vi "PicoScope3000aSettings.vi"(0 "handle in":i16, 1 "Channel A Settings":T1={"Enabled"=FALSE, "Coupling"=1, "Range"=6, "Analogue Offset"=0.0, "Bandwidth Limit"=0} {"Bandwidth Limit" items=["Full", "20MHz"]; "Range" items=["10 mV", "20 mV", "50 mV", "100 mV", "200 mV", "500 mV", "1 V", "2 V", "5 V", "10 V", "20 V", "50 V ", "100 V"]; "Coupling" items=["AC", "DC"]}, 2 "Channel B Settings":T1={"Enabled"=FALSE, "Coupling"=1, "Range"=6, "Analogue Offset"=0.0, "Bandwidth Limit"=0} {"Bandwidth Limit" items=["Full", "20MHz"]; "Range" items=["10 mV", "20 mV", "50 mV", "100 mV", "200 mV", "500 mV", "1 V", "2 V", "5 V", "10 V", "20 V", "50 V ", "100 V"]; "Coupling" items=["AC", "DC"]}, 3 "Port 0 Settings":T4={"Enabled"=FALSE, "Logic Level"=9830} {"Logic Level" items=["1.5V TTL"=9830, "2.5V CMOS"=16383]}, 5 "Trigger Settings":T3={"Trigger Enabled"=FALSE, "Trigger Source"=enum."Channel A", "Trigger Threshold (volts)"=0.0, "Trigger Direction"=2, "Trigger Delay (samples)"=0, "Auto Trigger Time (ms)"=1000} {"Trigger Direction" items=["Above", "Below", "Rising", "Falling", "Rising or Falling"]}, 7 "Max_adc":i16=32767, 9 "Device Info":T2, 11 "error in":errorcluster, 12 "Channel C Settings":T1={"Enabled"=FALSE, "Coupling"=1, "Range"=6, "Analogue Offset"=0.0, "Bandwidth Limit"=0} {"Bandwidth Limit" items=["Full", "20MHz"]; "Range" items=["10 mV", "20 mV", "50 mV", "100 mV", "200 mV", "500 mV", "1 V", "2 V", "5 V", "10 V", "20 V", "50 V ", "100 V"]; "Coupling" items=["AC", "DC"]}, 13 "Channel D Settings":T1={"Enabled"=FALSE, "Coupling"=1, "Range"=6, "Analogue Offset"=0.0, "Bandwidth Limit"=0} {"Bandwidth Limit" items=["Full", "20MHz"]; "Range" items=["10 mV", "20 mV", "50 mV", "100 mV", "200 mV", "500 mV", "1 V", "2 V", "5 V", "10 V", "20 V", "50 V ", "100 V"]; "Coupling" items=["AC", "DC"]}, 14 "Port 1 Settings":T4={"Enabled"=FALSE, "Logic Level"=9830} {"Logic Level" items=["1.5V TTL"=9830, "2.5V CMOS"=16383]}) -> (4 "handle out":i16, 8 "Enabled Array":i16[](array[numeric]), 15 "error out":errorcluster)   [LabVIEW 2010]
doc: "This VI is used to set up the oscilloscope channels and call the SetSimpleTrigger function."
uses:
  ps3000a.dll
  PicoScope3000aAnalogChannelSettings.ctl
  PicoScope3000aDigitalChannelSettings.ctl
panel:
  # "Connect to PicoScope3000aOpen.vi"
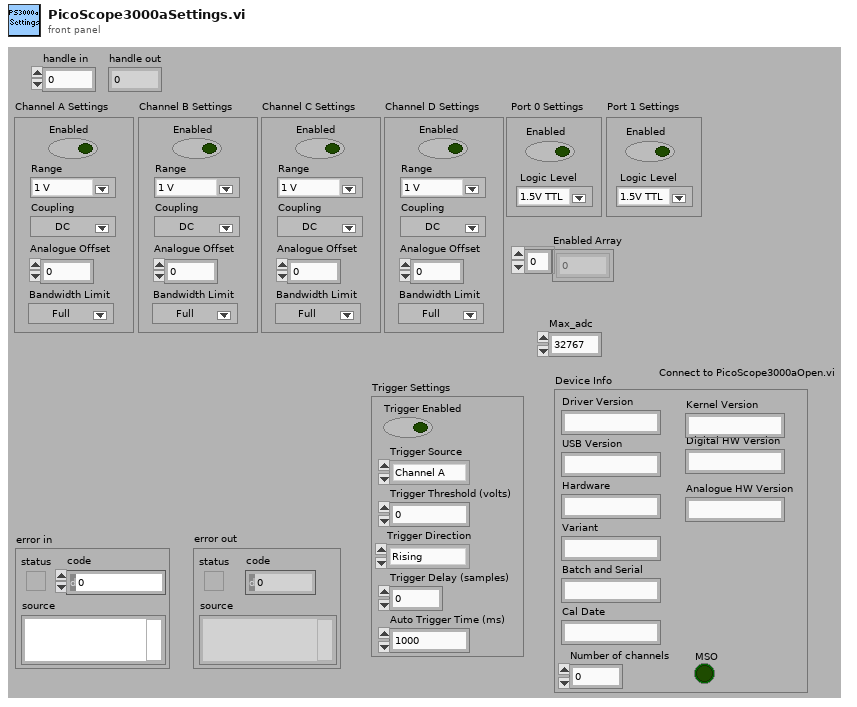
[diagram p1: front panel]
types:
  T1 = typedef "PicoScope3000aAnalogChannelSettings.ctl" = cluster{"Enabled":bool, "Coupling":u32, "Range":u32, "Analogue Offset":sgl, "Bandwidth Limit":u32}
  T2 = cluster{"Driver Version":string, "USB Version":string, "Hardware":string, "Variant":string, "Batch and Serial":string, "Cal Date":string, "Kernel Version":string, "Digital HW Version":string, "Analogue HW Version":string, "MSO":bool, "Number of channels":i16}
  T3 = cluster{"Trigger Enabled":bool, "Trigger Source":enum32{"Channel A", "Channel B", "Channel C", "Channel D", "Ext."}, "Trigger Threshold (volts)":dbl, "Trigger Direction":u32, "Trigger Delay (samples)":u32, "Auto Trigger Time (ms)":i16}
  T4 = typedef "PicoScope3000aDigitalChannelSettings.ctl" = cluster{"Enabled":bool, "Logic Level":i16}
  T5 = enum32{"Channel A", "Channel B", "Channel C", "Channel D", "Ext."}
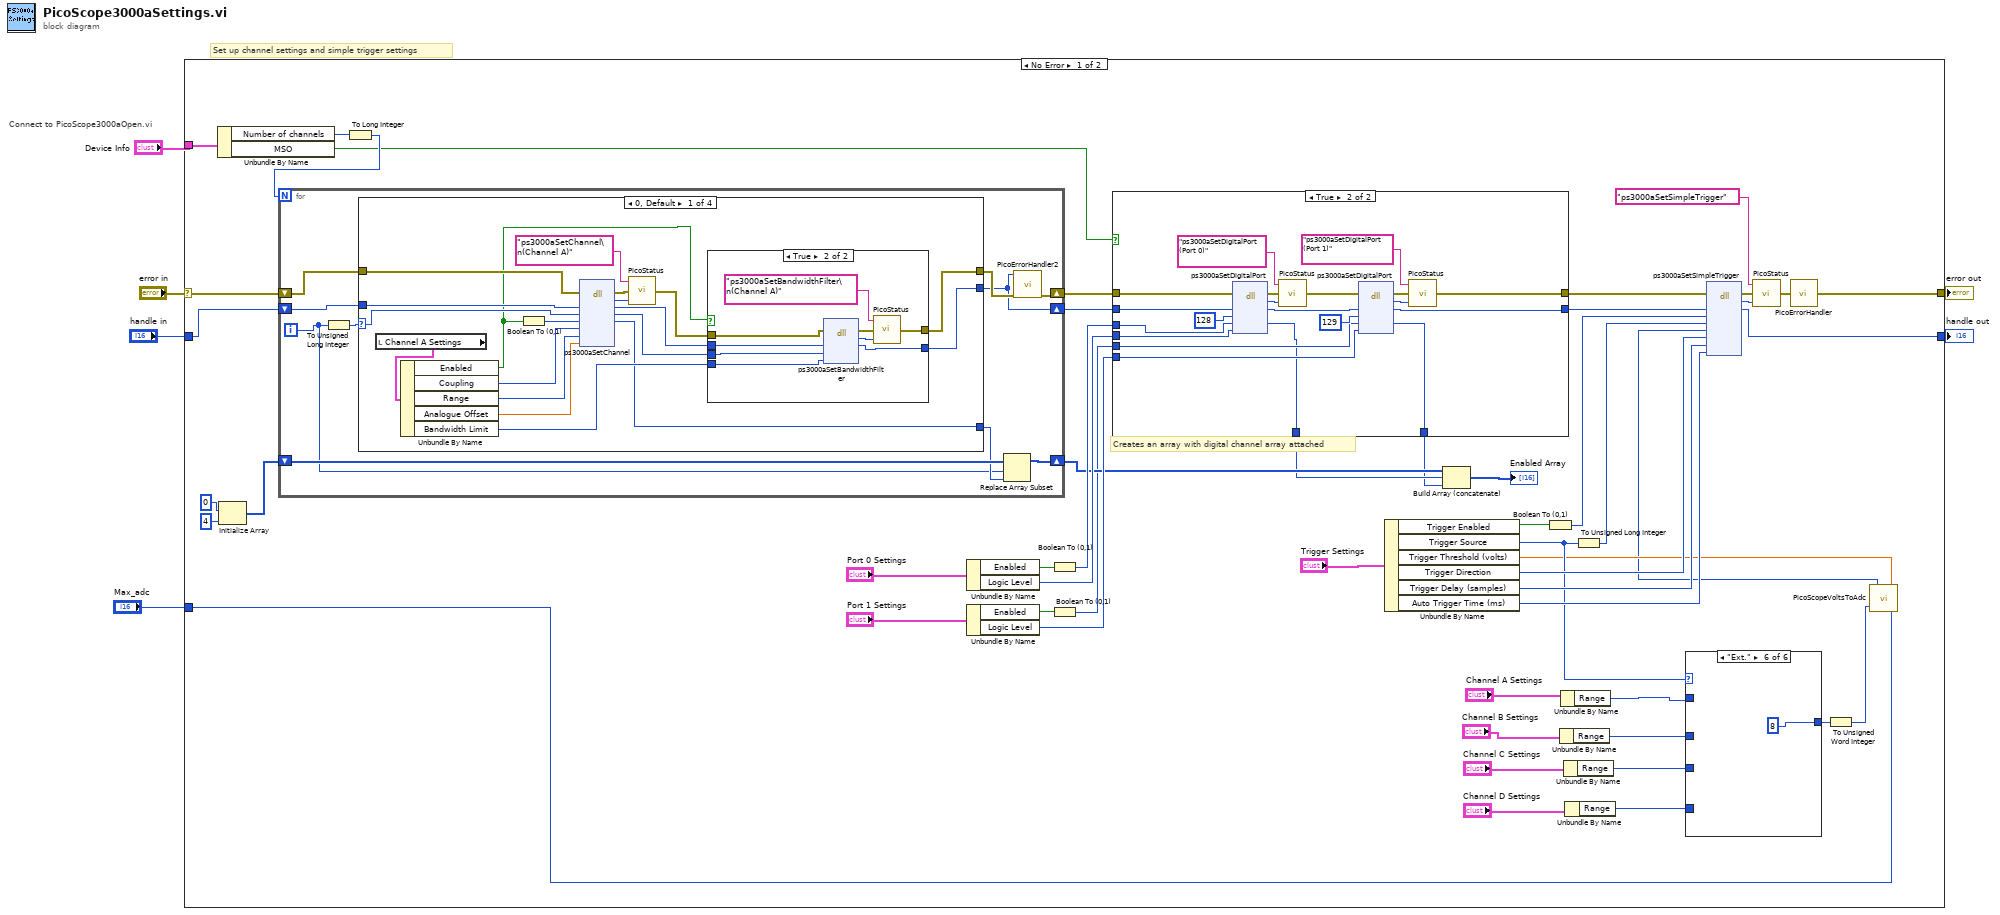
[diagram p0: block diagram]
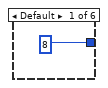
[diagram p2: hidden frame]
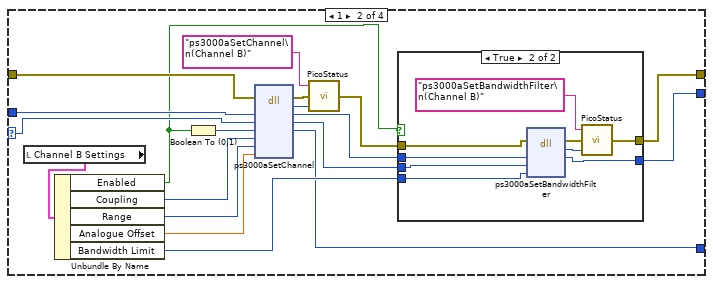
[diagram p8: hidden frame]
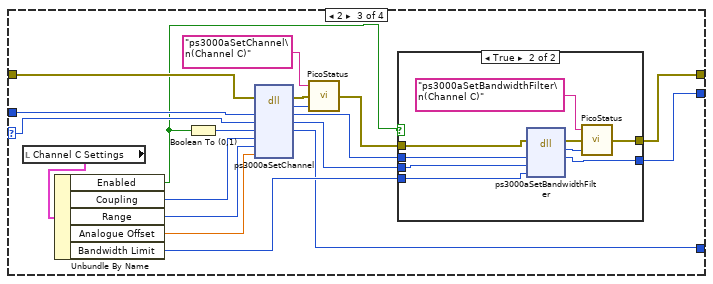
[diagram p10: hidden frame]
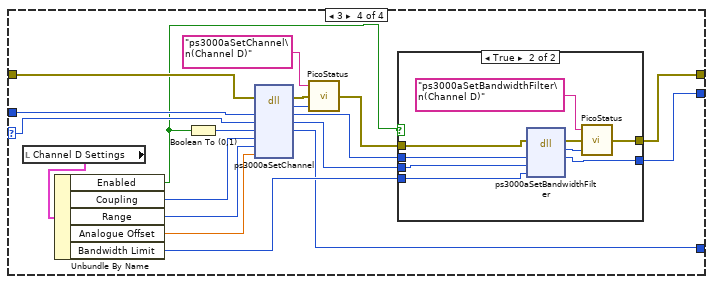
[diagram p12: hidden frame]
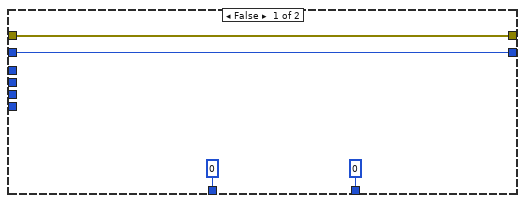
[diagram p14: hidden frame]
diagram:
  # "Connect to PicoScope3000aOpen.vi"
  # "Set up channel settings and simple trigger settings"
  n1 = case shown="No Error" "error in" {
    selector: "error in" -> [w39 w220]
    tunnel: "handle in" -> [w38 w219]
    tunnel: [w50 w219] -> w4
    tunnel: [w49 w220] -> w3
    tunnel: "Max_adc" -> [w7 _]
    tunnel: "Device Info" -> [w27 _]
    frame No Error {
      # "Creates an array with digital channel array attached"
      n2 = Unbundle By Name(w27) -> ("Number of channels"=w26:i16, "MSO"=w24:bool)
      n3 = Initialize Array(i16 0 ("element"), 4 ("dimension size")) -> (w31:i16[])
      n4 = To Long Integer(number=w26) -> (32bit integer=w25:i32)
      n5 = for {
        N: w25 -> [_]
        shift-right: [w69] -> w37
        shift-left: w39 -> [w74]
        shift-right: [w67] -> w36
        shift-left: w38 -> [w73]
        shift-right: [w72] -> w30
        shift-left: w31 -> [w71]
        i -> [w65]
        n6 = To Unsigned Long Integer(number=w65) -> (unsigned 32bit integer=w66:u32)
        n7 = case shown="0, Default" w66 {
          selector: w66 -> [w84 w114 w144 w174]
          tunnel: w74 -> [w93 w123 w153 w183]
          tunnel: [w78 w107 w137 w167] -> w68
          tunnel: w73 -> [w92 w122 w152 w182]
          tunnel: [w77 w106 w136 w166] -> w67
          tunnel: [w76 w105 w135 w165] -> w70
          frame 0, Default {
            n8 = local read "Channel A Settings"() -> (w75:T1)
            n9 = Unbundle By Name(w75) -> ("Enabled"=w79:bool, "Coupling"=w87:u32, "Range"=w86:u32, "Analogue Offset"=w85:sgl, "Bandwidth Limit"=w80:u32)
            n10 = Boolean To (0,1)(Boolean=w79) -> (0, 1=w88:i16)
            n11 = dll-call lib="ps3000a.dll" fn="ps3000aSetChannel" ("ps3000.dll:_ps3000_open_unit@0")(error in=w93, "handle"=w92, "channel"=w84, "enabled"=w88, "dc"=w87, "range"=w86, "analogueOffset"=w85) -> (error out=w90:errorcluster, "PICO_STATUS"=w91:u32, "handle"=w83:i16, "channel"=w81:u32, "enabled"=w76:i16)  [unwired: 5 in, 1 out]
            n12 = call "PicoStatus.vi"("PICO STATUS"=w91, "error in"=w90, "source"="ps3000aSetChannel\n(Channel A)") -> ("error out"=w82:errorcluster)
            n13 = case shown="True" w79 {
              tunnel: w83 -> [w94 w103]
              tunnel: w82 -> [w95 w102]
              tunnel: w81 -> [_ w101]
              tunnel: w80 -> [_ w100]
              tunnel: [w95 w99] -> w78
              tunnel: [w94 w96] -> w77
              frame False {
              }
              frame True {
                n14 = dll-call lib="ps3000a.dll" fn="ps3000aSetBandwidthFilter" ("ps3000.dll:_ps3000_open_unit@0")(error in=w102, "handle"=w103, "channel"=w101, "bandwidth"=w100) -> (error out=w104:errorcluster, "PICO_STATUS"=w98:u32, "handle"=w96:i16)  [unwired: 4 in, 1 out]
                n15 = call "PicoStatus.vi"("PICO STATUS"=w98, "error in"=w104, "source"="ps3000aSetBandwidthFilter\n(Channel A)") -> ("error out"=w99:errorcluster)
              }
            }
          }
          frame 1 {
            n16 = local read "Channel B Settings"() -> (w113:T1)
            n17 = Unbundle By Name(w113) -> ("Enabled"=w108:bool, "Coupling"=w117:u32, "Range"=w116:u32, "Analogue Offset"=w115:sgl, "Bandwidth Limit"=w109:u32)
            n18 = Boolean To (0,1)(Boolean=w108) -> (0, 1=w118:i16)
            n19 = dll-call lib="ps3000a.dll" fn="ps3000aSetChannel" ("ps3000.dll:_ps3000_open_unit@0")(error in=w123, "handle"=w122, "channel"=w114, "enabled"=w118, "dc"=w117, "range"=w116, "analogueOffset"=w115) -> (error out=w120:errorcluster, "PICO_STATUS"=w121:u32, "handle"=w112:i16, "channel"=w110:u32, "enabled"=w105:i16)  [unwired: 5 in, 1 out]
            n20 = call "PicoStatus.vi"("PICO STATUS"=w121, "error in"=w120, "source"="ps3000aSetChannel\n(Channel B)") -> ("error out"=w111:errorcluster)
            n21 = case shown="True" w108 {
              tunnel: w112 -> [w124 w133]
              tunnel: w111 -> [w125 w132]
              tunnel: w110 -> [_ w131]
              tunnel: w109 -> [_ w130]
              tunnel: [w125 w129] -> w107
              tunnel: [w124 w126] -> w106
              frame False {
              }
              frame True {
                n22 = dll-call lib="ps3000a.dll" fn="ps3000aSetBandwidthFilter" ("ps3000.dll:_ps3000_open_unit@0")(error in=w132, "handle"=w133, "channel"=w131, "bandwidth"=w130) -> (error out=w134:errorcluster, "PICO_STATUS"=w128:u32, "handle"=w126:i16)  [unwired: 4 in, 1 out]
                n23 = call "PicoStatus.vi"("PICO STATUS"=w128, "error in"=w134, "source"="ps3000aSetBandwidthFilter\n(Channel B)") -> ("error out"=w129:errorcluster)
              }
            }
          }
          frame 2 {
            n24 = local read "Channel C Settings"() -> (w143:T1)
            n25 = Unbundle By Name(w143) -> ("Enabled"=w138:bool, "Coupling"=w147:u32, "Range"=w146:u32, "Analogue Offset"=w145:sgl, "Bandwidth Limit"=w139:u32)
            n26 = Boolean To (0,1)(Boolean=w138) -> (0, 1=w148:i16)
            n27 = dll-call lib="ps3000a.dll" fn="ps3000aSetChannel" ("ps3000.dll:_ps3000_open_unit@0")(error in=w153, "handle"=w152, "channel"=w144, "enabled"=w148, "dc"=w147, "range"=w146, "analogueOffset"=w145) -> (error out=w150:errorcluster, "PICO_STATUS"=w151:u32, "handle"=w142:i16, "channel"=w140:u32, "enabled"=w135:i16)  [unwired: 5 in, 1 out]
            n28 = call "PicoStatus.vi"("PICO STATUS"=w151, "error in"=w150, "source"="ps3000aSetChannel\n(Channel C)") -> ("error out"=w141:errorcluster)
            n29 = case shown="True" w138 {
              tunnel: w142 -> [w154 w163]
              tunnel: w141 -> [w155 w162]
              tunnel: w140 -> [_ w161]
              tunnel: w139 -> [_ w160]
              tunnel: [w155 w159] -> w137
              tunnel: [w154 w156] -> w136
              frame False {
              }
              frame True {
                n30 = dll-call lib="ps3000a.dll" fn="ps3000aSetBandwidthFilter" ("ps3000.dll:_ps3000_open_unit@0")(error in=w162, "handle"=w163, "channel"=w161, "bandwidth"=w160) -> (error out=w164:errorcluster, "PICO_STATUS"=w158:u32, "handle"=w156:i16)  [unwired: 4 in, 1 out]
                n31 = call "PicoStatus.vi"("PICO STATUS"=w158, "error in"=w164, "source"="ps3000aSetBandwidthFilter\n(Channel C)") -> ("error out"=w159:errorcluster)
              }
            }
          }
          frame 3 {
            n32 = local read "Channel D Settings"() -> (w173:T1)
            n33 = Unbundle By Name(w173) -> ("Enabled"=w168:bool, "Coupling"=w177:u32, "Range"=w176:u32, "Analogue Offset"=w175:sgl, "Bandwidth Limit"=w169:u32)
            n34 = Boolean To (0,1)(Boolean=w168) -> (0, 1=w178:i16)
            n35 = dll-call lib="ps3000a.dll" fn="ps3000aSetChannel" ("ps3000.dll:_ps3000_open_unit@0")(error in=w183, "handle"=w182, "channel"=w174, "enabled"=w178, "dc"=w177, "range"=w176, "analogueOffset"=w175) -> (error out=w180:errorcluster, "PICO_STATUS"=w181:u32, "handle"=w172:i16, "channel"=w170:u32, "enabled"=w165:i16)  [unwired: 5 in, 1 out]
            n36 = call "PicoStatus.vi"("PICO STATUS"=w181, "error in"=w180, "source"="ps3000aSetChannel\n(Channel D)") -> ("error out"=w171:errorcluster)
            n37 = case shown="True" w168 {
              tunnel: w172 -> [w184 w193]
              tunnel: w171 -> [w185 w192]
              tunnel: w170 -> [_ w191]
              tunnel: w169 -> [_ w190]
              tunnel: [w185 w189] -> w167
              tunnel: [w184 w186] -> w166
              frame False {
              }
              frame True {
                n38 = dll-call lib="ps3000a.dll" fn="ps3000aSetBandwidthFilter" ("ps3000.dll:_ps3000_open_unit@0")(error in=w192, "handle"=w193, "channel"=w191, "bandwidth"=w190) -> (error out=w194:errorcluster, "PICO_STATUS"=w188:u32, "handle"=w186:i16)  [unwired: 4 in, 1 out]
                n39 = call "PicoStatus.vi"("PICO STATUS"=w188, "error in"=w194, "source"="ps3000aSetBandwidthFilter\n(Channel D)") -> ("error out"=w189:errorcluster)
              }
            }
          }
        }
        n40 = Replace Array Subset(array=w71, new element=w70, index=w65) -> (w72:i16[])
        n41 = call "PicoErrorHandler2.vi"("error in (no error)"=w68, "handle In"=w67) -> ("error out"=w69:errorcluster)  [unwired: 9 in]
      }
      n42 = Unbundle By Name("Port 0 Settings") -> ("Enabled"=w47:bool, "Logic Level"=w46:i16)
      n43 = Unbundle By Name("Port 1 Settings") -> ("Enabled"=w44:bool, "Logic Level"=w43:i16)
      n44 = Boolean To (0,1)(Boolean=w47) -> (0, 1=w34:i16)
      n45 = Boolean To (0,1)(Boolean=w44) -> (0, 1=w29:i16)
      n46 = case shown="True" w24 {
        tunnel: w36 -> [w197 w218]
        tunnel: w34 -> [_ w216]
        tunnel: w46 -> [_ w215]
        tunnel: w29 -> [_ w206]
        tunnel: w43 -> [_ w205]
        tunnel: [w197 w211] -> w42
        tunnel: [w198 w208] -> w41
        tunnel: w37 -> [w198 w204]
        tunnel: [i16 0 ("enabled") w200] -> w12
        tunnel: [i16 0 ("enabled") w199] -> w11
        frame False {
        }
        frame True {
          n47 = dll-call lib="PS3000a.dll" fn="ps3000aSetDigitalPort"(error in=w204, "handle"=w218, "port"=u32 128, "enabled"=w216, "logicLevel"=w215) -> (error out=w214:errorcluster, "PICO_STATUS"=w202:u32, "handle"=w212:i16, "enabled"=w200:i16)  [unwired: 4 in, 1 out]
          n48 = call "PicoStatus.vi"("PICO STATUS"=w202, "error in"=w214, "source"="ps3000aSetDigitalPort (Port 0)") -> ("error out"=w203:errorcluster)
          n49 = dll-call lib="PS3000a.dll" fn="ps3000aSetDigitalPort"(error in=w203, "handle"=w212, "port"=u32 129, "enabled"=w206, "logicLevel"=w205) -> (error out=w213:errorcluster, "PICO_STATUS"=w201:u32, "handle"=w211:i16, "enabled"=w199:i16)  [unwired: 4 in, 1 out]
          n50 = call "PicoStatus.vi"("PICO STATUS"=w201, "error in"=w213, "source"="ps3000aSetDigitalPort (Port 1)") -> ("error out"=w208:errorcluster)
        }
      }
      n51 = Unbundle By Name("Trigger Settings") -> ("Trigger Enabled"=w56:bool, "Trigger Source"=w23:T5, "Trigger Threshold (volts)"=w22:dbl, "Trigger Direction"=w40:u32, "Trigger Delay (samples)"=w58:u32, "Auto Trigger Time (ms)"=w57:i16)
      n52 = Build Array (concatenate)(w30, w12, w11) -> (→"Enabled Array":i16[])
      n53 = Boolean To (0,1)(Boolean=w56) -> (0, 1=w55:i16)
      n54 = Unbundle By Name("Channel B Settings") -> ("Range"=w19:u32)
      n55 = Unbundle By Name("Channel A Settings") -> ("Range"=w16:u32)
      n56 = Unbundle By Name("Channel C Settings") -> ("Range"=w18:u32)
      n57 = Unbundle By Name("Channel D Settings") -> ("Range"=w17:u32)
      n58 = To Unsigned Long Integer(number=w23) -> (unsigned 32bit integer=w35:u32)
      n59 = case shown="\"Ext.\"" w23 {
        tunnel: w16 -> [_ w60 _ _ _ _]
        tunnel: w19 -> [_ _ w61 _ _ _]
        tunnel: w18 -> [_ _ _ w62 _ _]
        tunnel: w17 -> [_ _ _ _ w63 _]
        tunnel: [u32 8 ("Range") w60 w61 w62 w63 u32 8] -> w14
        frame Default {
        }
        frame "Channel A" {
        }
        frame "Channel B" {
        }
        frame "Channel C" {
        }
        frame "Channel D" {
        }
        frame "Ext." {
        }
      }
      n60 = To Unsigned Word Integer(number=w14) -> (unsigned 16bit integer=w15:u16)
      n61 = call "PicoScopeVoltsToAdc.vi"("Max_adc"=w7, "Volts"=w22, "Range Index"=w15) -> ("ADC count"=w21:i16)
      n62 = dll-call lib="ps3000a.dll" fn="ps3000aSetSimpleTrigger" ("ps3000.dll:_ps3000_open_unit@0")(error in=w41, "handle"=w42, "enabled"=w55, "source"=w35, "threshold"=w21, "direction"=w40, "delay"=w58, "autoTrigger_ms"=w57) -> (error out=w53:errorcluster, "PICO_STATUS"=w54:u32, "handle"=w50:i16)  [unwired: 8 in, 1 out]
      n63 = call "PicoStatus.vi"("PICO STATUS"=w54, "error in"=w53, "source"="ps3000aSetSimpleTrigger") -> ("error out"=w51:errorcluster)
      n64 = call "PicoErrorHandler.vi"("error in"=w51) -> ("error out"=w49:errorcluster)
    }
    frame Error {
    }
  }
  "handle out" <- w4
  "error out" <- w3
